vi "Build VIH Deployment.vi"(4 "Exclude file name patterns":string, 6 "Folders":string="Examples\nHelp\nProject\nvi.lib", 7 "Exclude undesired paths (T)":bool=TRUE, 8 "error in":errorcluster, 9 "LV Version":string(combo)="14.0", 10 "Target Dir":path, 11 "Source Dir":path) -> (0 "error out":errorcluster, 1 "Excluded Paths":path[](array[path]), 2 "dup Target Dir":path, 3 "dup Source Dir":path)   [LabVIEW 2014]
doc: "::: VI Helpeks :::\nCopyright (c) 2000-2026 Konstantin Shifershteyn. All rights reserved."
panel:
  # "VI Helpeks\nCopyright (c) 2012-2026 Konstantin Shifershteyn"
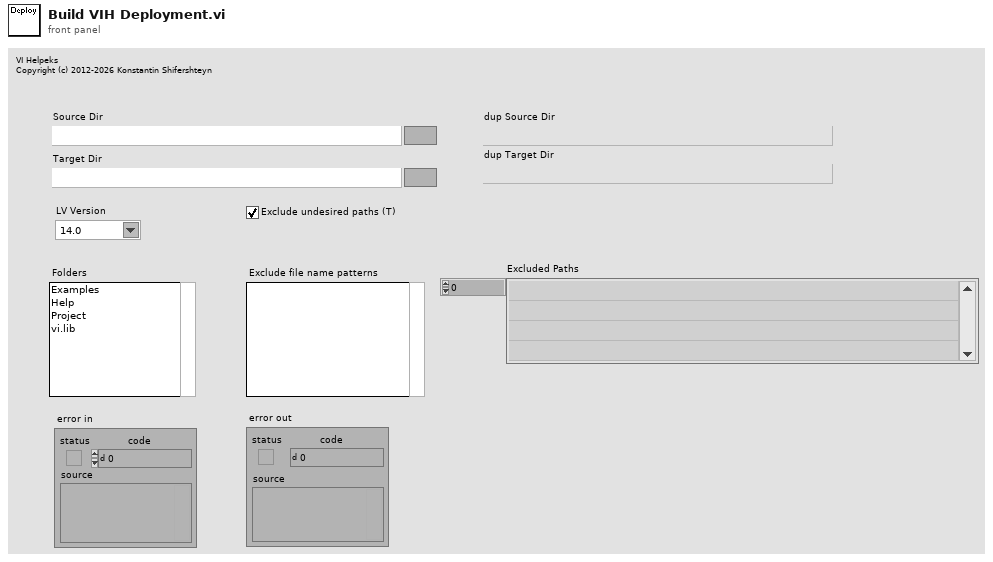
[diagram p1: front panel]
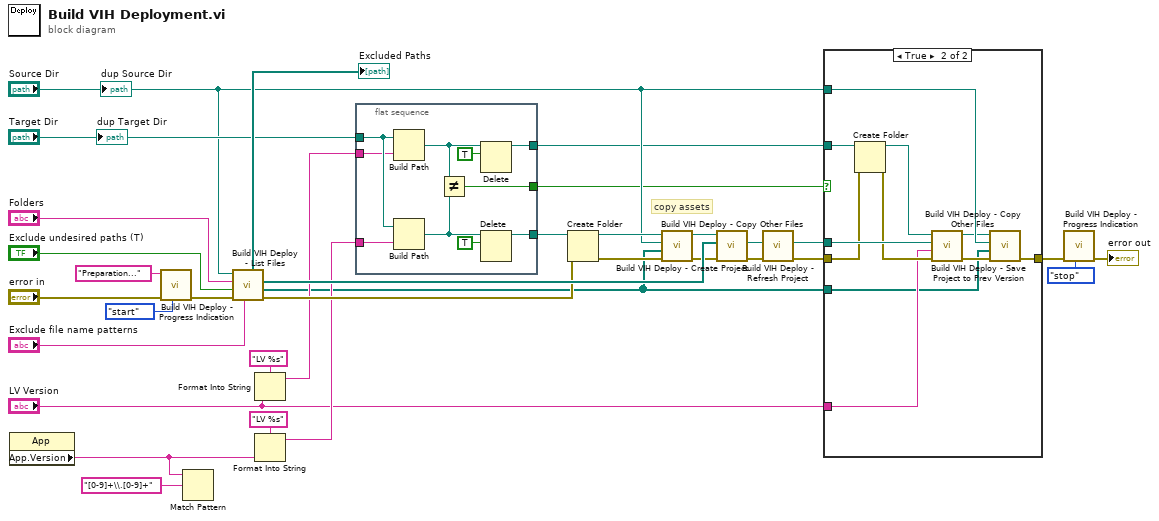
[diagram p0: block diagram]
diagram:
  # "copy assets"
  n1 = property class="App"() -> ("App.Version"=w12:string)  [unwired: 2 in, 2 out]
  n2 = call "Build VIH Deploy - Progress Indication.vi"("mode (run)"=enum16{"run", "start", "stop"}."start", "error in"="error in", "message 1"="Preparation...") -> ("error out"=w21:errorcluster)  [unwired: 8 in]
  n3 = Match Pattern(string=w12, regular expression="[0-9]+\\.[0-9]+") -> ()  [unwired: 1 in, 4 out]
  n4 = call "Build VIH Deploy - List Files.vi"("Exclude file names"="Exclude file name patterns", "error in"=w21, "Exclude undesired paths (F)"="Exclude undesired paths (T)", "Folders"="Folders", "Source Dir"="Source Dir") -> ("error out"=w25:errorcluster, "Files to Copy"=w4:path[], "Project Files"=w34:path[], "Excluded Paths"=→"Excluded Paths":path[])  [unwired: 2 in, 1 out]
  n5 = Format Into String(format string="LV %s", "LV Version") -> (resulting string=w9:string)  [unwired: 2 in, 1 out]
  n6 = Format Into String(format string="LV %s", w12) -> (resulting string=w11:string)  [unwired: 2 in, 1 out]
  n7 = flat-sequence {
    tunnel: [w44] -> w26
    tunnel: w11 -> [w42]
    tunnel: "Target Dir" -> [w41]
    tunnel: w9 -> [w40]
    tunnel: [w38] -> w2
    tunnel: [w35] -> w1
    frame #0 {
      n8 = Build Path(base path=w41, name or relative path=w40) -> (appended path=w36:path)
      n9 = Build Path(base path=w41, name or relative path=w42) -> (appended path=w39:path)
      n10 = Not Equal?(x=w36, y=w39) -> (x != y?=w38:bool)
      n11 = Delete(path (use dialog)=w36, entire hierarchy (F)=TRUE) -> (deleted path=w35:path)  [unwired: 3 in, 2 out]
      n12 = Delete(path (use dialog)=w39, entire hierarchy (F)=TRUE) -> (deleted path=w44:path)  [unwired: 3 in, 2 out]
    }
  }
  n13 = Create Folder(path (use dialog)=w26, error in=w25) -> (created path=w24:path, error out=w17:errorcluster)  [unwired: 1 in, 1 out]
  n14 = call "Build VIH Deploy - Copy Other Files.vi"("error in"=w17, "Files to Copy"=w4, "Source Dir"="Source Dir", "Target Dir"=w24) -> ("error out"=w29:errorcluster, "dup Target Dir"=w30:path)  [unwired: 6 in]
  n15 = call "Build VIH Deploy - Create Project.vi"("error in"=w29, "Project Files"=w34, "Target Dir"=w30) -> ("error out"=w16:errorcluster, "Project File Path"=w15:path)  [unwired: 6 in, 1 out]
  n16 = call "Build VIH Deploy - Refresh Project.vi"("error in"=w16, "Project file"=w15) -> ("error out"=w7:errorcluster, "dup Project file"=w8:path)  [unwired: 8 in]
  n17 = case shown="True" w2 {
    tunnel: w1 -> [_ w46]
    tunnel: w8 -> [_ w56]
    tunnel: w7 -> [w45 w54]
    tunnel: "LV Version" -> [_ w52]
    tunnel: [w45 w50] -> w5
    tunnel: w4 -> [_ w49]
    tunnel: "Source Dir" -> [_ w48]
    frame False {
    }
    frame True {
      n18 = Create Folder(path (use dialog)=w46, error in=w54) -> (created path=w55:path, error out=w53:errorcluster)  [unwired: 1 in, 1 out]
      n19 = call "Build VIH Deploy - Save Project to Prev Version.vi"("error in"=w53, "LV Version"=w52, "Project file"=w56, "Target Dir"=w55) -> ("error out"=w51:errorcluster, "dup Target Dir"=w47:path)  [unwired: 6 in]
      n20 = call "Build VIH Deploy - Copy Other Files.vi"("error in"=w51, "Files to Copy"=w49, "Source Dir"=w48, "Target Dir"=w47) -> ("error out"=w50:errorcluster)  [unwired: 6 in, 1 out]
    }
  }
  n21 = call "Build VIH Deploy - Progress Indication.vi"("mode (run)"=enum16{"run", "start", "stop"}."stop", "error in"=w5) -> ("error out"=→"error out":errorcluster)  [unwired: 9 in]
  "dup Target Dir" <- "Target Dir"
  "dup Source Dir" <- "Source Dir"
